vi "Add ECAT Variable Contents.vi"(5 "Name Prefix":string, 7 "Add Name Property":bool, 8 "error in":errorcluster, 9 "Input Parent Ref in":T1 format="%.0x", 10 "Output Parent Ref in":T1 format="%.0x", 11 "IO Variable Container Contents":T2) -> (0 "error out":errorcluster)   [LabVIEW 2020, in "SEECD System Explorer.lvlib"]
uses:
  SEECD System Explorer.lvlib
  Type Defs/IOV Container Contents.ctl
  <vilib>/NI VeriStand/Custom Device API/Custom Device Item Ref.ctl
  <vilib>/NI VeriStand/Custom Device API/Custom Device Channel.ctl
  <vilib>/NI VeriStand/Custom Device API/Custom Device Channel Type.ctl
  Shared/Globals/Property Strings.vi
  Shared/Globals/Scan Engine GUIDs.vi
  <vilib>/NI VeriStand/Custom Device API/Set Item Property (String).vi
  <vilib>/NI VeriStand/Custom Device API/Custom Device API.lvlib
  Shared/SEECD Shared.lvlib
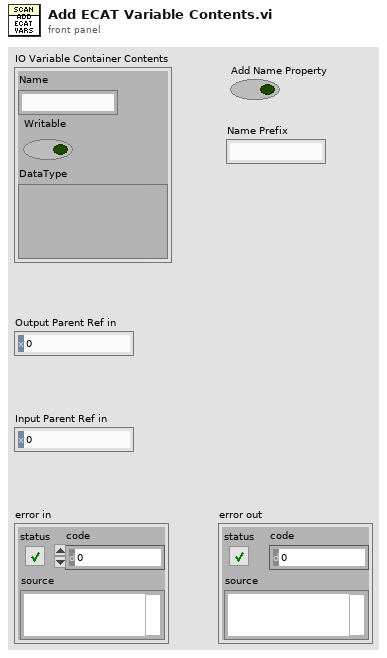
[diagram p1: front panel]
types:
  T1 = typedef "Custom Device API.lvlib/Custom Device Item Ref.ctl" = u64
  T2 = typedef "SEECD System Explorer.lvlib/IOV Container Contents.ctl" = cluster{"Name":string, "Writable":bool, "DataType":variant}
  T3 = typedef "Custom Device API.lvlib/Custom Device Channel.ctl" = cluster{"Type":T4, "Units":string, "Default Value":dbl, "Faultable":bool, "Scalable":bool}
  T4 = typedef "Custom Device API.lvlib/Custom Device Channel Type.ctl" = enum16{"Input", "Output"}
  T5 = typedef "SEECD Shared.lvlib/ECAT Channel Data Type.ctl" = enum16{"Boolean", "Fixed Point", "Int8", "Int16", "Int32", "Int64", "U32 Bit Field", "UInt8", "UInt16", "UInt32", "UInt64", "Other", "DBL", "SGL"}
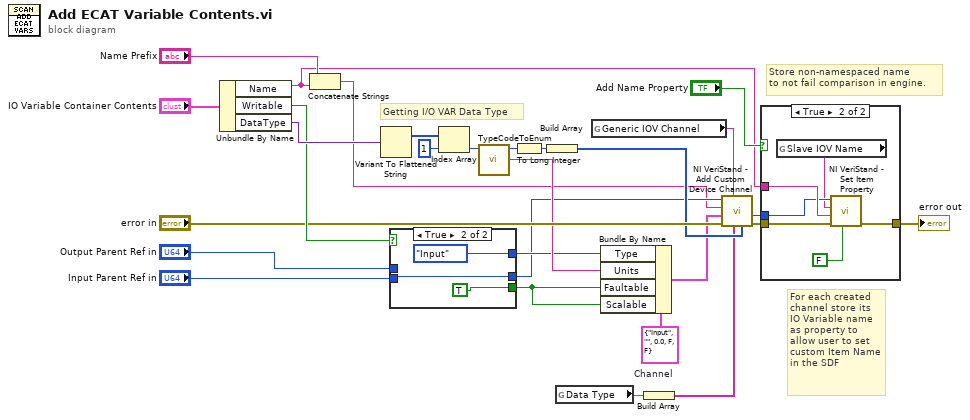
[diagram p0: block diagram]
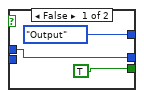
[diagram p3: hidden frame]
diagram:
  w5 = T3 {"Type"=enum."Input", "Units"="", "Default Value"=0.0, "Faultable"=FALSE, "Scalable"=FALSE}  # Channel
  # "Store non-namespaced name\nto not fail comparison in engine."
  # "For each created channel store its IO Variable name as property to allow user to set custom Item Name in the SDF"
  # "Getting I/O VAR Data Type"
  n1 = Unbundle By Name("IO Variable Container Contents") -> ("Name"=w1:string, "Writable"=w27:bool, "DataType"=w28:variant)
  n2 = Concatenate Strings("Name Prefix", w1) -> (w3:string)
  n3 = Variant To Flattened String(Variant=w28) -> (1:w8:i16[])  [unwired: 1 out]
  n4 = case shown="True" w27 {
    tunnel: [Custom_Device_Channel_Type."Output" ("Type") Custom_Device_Channel_Type."Input" ("Type")] -> w16
    tunnel: [w29 w32] -> w11
    tunnel: "Output Parent Ref in" -> [w29 _]
    tunnel: "Input Parent Ref in" -> [_ w32]
    tunnel: [TRUE TRUE] -> w13
    frame False {
    }
    frame True {
    }
  }
  n5 = Index Array(array=w8, index=1) -> (element=w18:i16)
  n6 = call "TypeCodeToEnum.vi"("Type Code (numbers in hexadecimal)"=w18) -> (2:"UDV Data Type"=w17:string, 3:"UDV Data Type"=w20:T5)  [unwired: 9 in]
  n7 = To Long Integer(number=w20) -> (32bit integer=w19:i32)
  n8 = Build Array(w19) -> (w15:i32[])
  n9 = global read "Property Strings.vi" "Data Type"() -> (w14:string)
  n10 = global read "Scan Engine GUIDs.vi" "Generic IOV Channel"() -> (w21:string)
  n11 = Bundle By Name(cluster=w5, "Type"=w16, "Units"=w17, "Faultable"=w13, "Scalable"=w13) -> (w6:T3)
  n12 = Build Array(w14) -> (w7:string[])
  n13 = call <vilib>:"NI VeriStand - Add Custom Device Channel.vi"("Property Values"=w15, "Property names"=w7, "GUID (Default Channel)"=w21, "error in (no error)"="error in", "Channel"=w6, "Channel Name"=w3, "Parent Ref in"=w11) -> ("error out"=w22:errorcluster, "Channel Ref"=w24:T1)  [unwired: 1 in, 2 out]
  n14 = case shown="True" "Add Name Property" {
    tunnel: w1 -> [_ w41]
    tunnel: w24 -> [_ w40]
    tunnel: [w35 w37] -> w23
    tunnel: w22 -> [w35 w36]
    frame False {
    }
    frame True {
      n15 = global read "Property Strings.vi" "Slave IOV Name"() -> (w39:string)
      n16 = call-poly <vilib>:"NI VeriStand - Set Item Property.vi"("Binary String (T)"=FALSE, "error in (no error)"=w36, "Value"=w41, "Property Name"=w39, "Item Ref in"=w40) -> ("error out"=w37:errorcluster)  [unwired: 4 in, 2 out]
    }
  }
  "error out" <- w23
